vi "Pre-Uninstall Custom Action.vi"(10 "Variant":variant) -> (0 "error out":errorcluster)   [LabVIEW 2014]
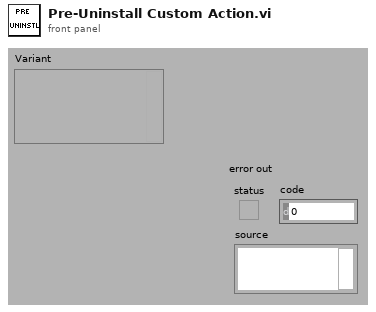
[diagram p1: front panel]
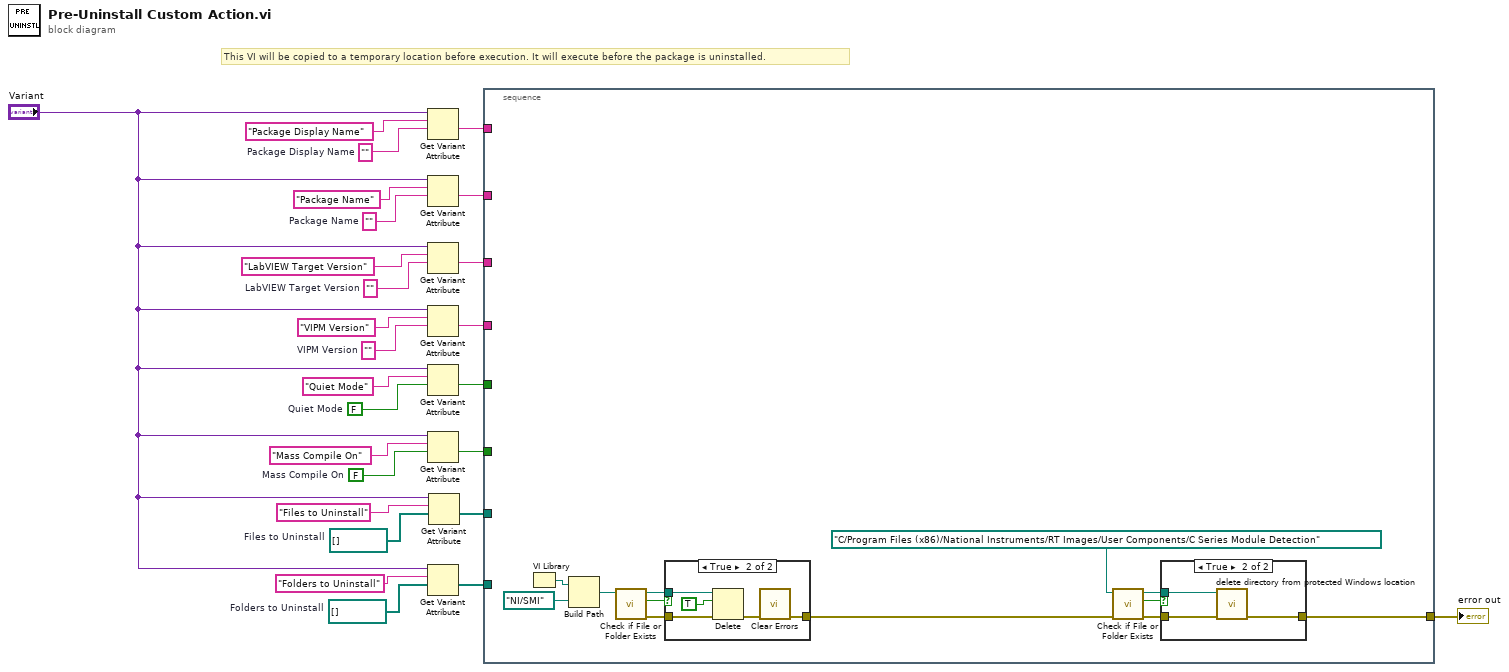
[diagram p0: block diagram]
diagram:
  w4 = path[] []  # Folders to Uninstall
  w8 = path[] []  # Files to Uninstall
  w9 = FALSE  # Mass Compile On
  w10 = ""  # Package Display Name
  w17 = FALSE  # Quiet Mode
  w20 = ""  # VIPM Version
  w22 = ""  # LabVIEW Target Version
  w24 = ""  # Package Name
  # "This VI will be copied to a temporary location before execution. It will execute before the package is uninstalled."
  n1 = Get Variant Attribute(Variant="Variant", name="Package Display Name", default value (empty Variant)=w10) -> (value=w16:string)  [unwired: 1 in, 3 out]
  n2 = Get Variant Attribute(Variant="Variant", name="Package Name", default value (empty Variant)=w24) -> (value=w15:string)  [unwired: 1 in, 3 out]
  n3 = Get Variant Attribute(Variant="Variant", name="LabVIEW Target Version", default value (empty Variant)=w22) -> (value=w14:string)  [unwired: 1 in, 3 out]
  n4 = Get Variant Attribute(Variant="Variant", name="VIPM Version", default value (empty Variant)=w20) -> (value=w13:string)  [unwired: 1 in, 3 out]
  n5 = Get Variant Attribute(Variant="Variant", name="Quiet Mode", default value (empty Variant)=w17) -> (value=w12:bool)  [unwired: 1 in, 3 out]
  n6 = Get Variant Attribute(Variant="Variant", name="Mass Compile On", default value (empty Variant)=w9) -> (value=w11:bool)  [unwired: 1 in, 3 out]
  n7 = Get Variant Attribute(Variant="Variant", name="Folders to Uninstall", default value (empty Variant)=w4) -> (value=w3:path[])  [unwired: 1 in, 3 out]
  n8 = Get Variant Attribute(Variant="Variant", name="Files to Uninstall", default value (empty Variant)=w8) -> (value=w6:path[])  [unwired: 1 in, 3 out]
  n9 = stacked-sequence {
    tunnel: w16 -> [_]
    tunnel: w15 -> [_]
    tunnel: w14 -> [_]
    tunnel: w13 -> [_]
    tunnel: w12 -> [_]
    tunnel: w11 -> [_]
    tunnel: w6 -> [_]
    tunnel: w3 -> [_]
    tunnel: [w27] -> w1
    frame #0 {
      n10 = VI Library() -> (path=w28:path)
      n11 = Build Path(base path=w28, name or relative path=path "NI/SMI") -> (appended path=w30:path)
      n12 = call <vilib>:"Check if File or Folder Exists.vi"("path"=w30) -> ("error out"=w32:errorcluster, "file or folder exists?"=w33:bool, "dup path"=w31:path)  [unwired: 8 in]
      n13 = case shown="True" w33 {
        tunnel: [w43 w46] -> w35
        tunnel: w31 -> [_ w45]
        tunnel: w32 -> [w43 w44]
        frame False {
        }
        frame True {
          n14 = Delete(path (use dialog)=w45, entire hierarchy (F)=TRUE, error in=w44) -> (error out=w47:errorcluster)  [unwired: 2 in, 2 out]
          n15 = call <vilib>:"Clear Errors.vi"("error in (no error)"=w47) -> ("error out"=w46:errorcluster)  [unwired: 5 in, 1 out]
        }
      }
      n16 = call <vilib>:"Check if File or Folder Exists.vi"("error in (no error)"=w35, "path"=path "C:/Program Files (x86)/National Instruments/RT Images/User Components/C Series Module Detection" ("directory")) -> ("error out"=w37:errorcluster, "file or folder exists?"=w36:bool, "dup path"=w38:path)  [unwired: 7 in]
      n17 = case shown="True" w36 {
        tunnel: w37 -> [w39 w42]
        tunnel: [w39 w41] -> w27
        tunnel: w38 -> [_ w40]
        frame False {
        }
        frame True {
          n18 = call "delete directory from protected Windows location.vi"("error in"=w42, "directory"=w40) -> ("error out"=w41:errorcluster)  [unwired: 8 in, 1 out]
        }
      }
    }
  }
  "error out" <- w1
